vi "set Swept SA - Marker.vi"(6 "On?":bool, 8 "error in (no error)":errorcluster, 9 "trace":i32, 10 "Index":i32, 11 "Keysight 9020A in":refnum<class "Keysight 9020A.lvclass">) -> (0 "error out":errorcluster, 3 "Keysight 9020A out":refnum<class "Keysight 9020A.lvclass">)   [LabVIEW 2023, in "Spectrum Analyzer.lvlib" / "Keysight 9020A.lvclass"]
uses:
  Keysight 9020A.lvclass
  Keysight 9020A.lvclass/Keysight 9020A.ctl
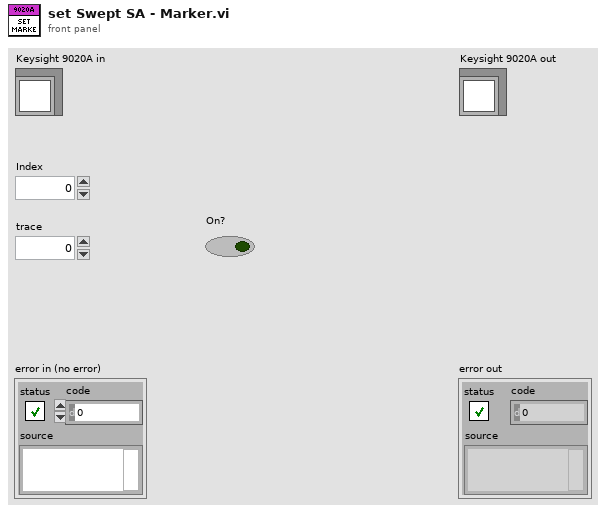
[diagram p1: front panel]
types:
  T1 = typedef "Spectrum Analyzer.lvlib/TYPE Measurement Preset.ctl" = enum16{"Sweep SA Mode", "Channel Power", "Occupied BW", "ACP", "Spurious Emission", "Spurious Emission Mask", "Burst Power (Transmit Power)"}
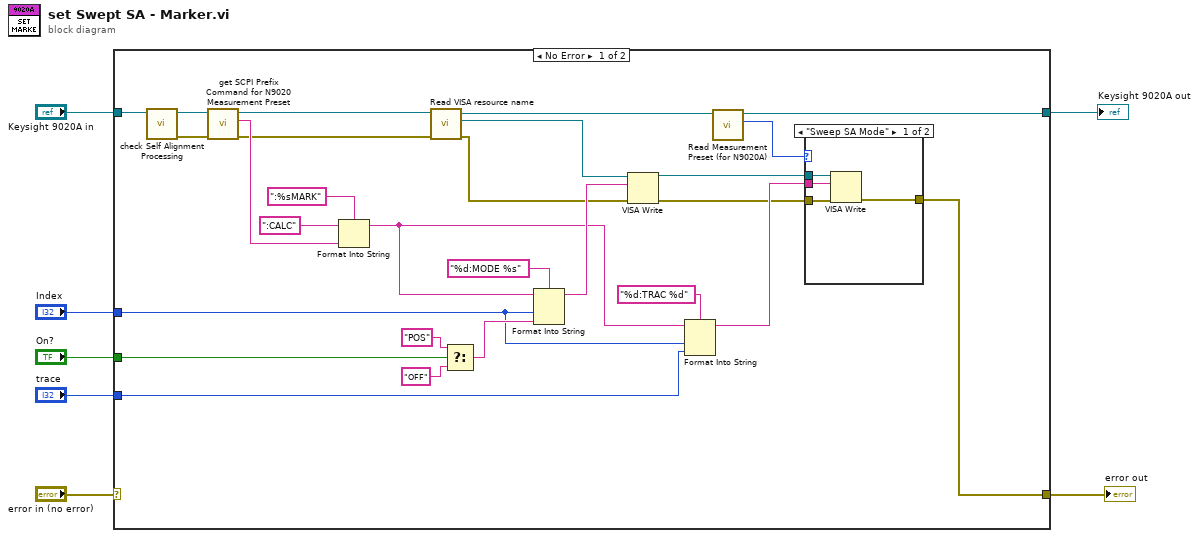
[diagram p0: block diagram]
diagram:
  n1 = case shown="No Error" "error in (no error)" {
    selector: "error in (no error)" -> [_ w40]
    tunnel: "Keysight 9020A in" -> [w12 w41]
    tunnel: [w14 w41] -> w6
    tunnel: [w22 w40] -> w4
    tunnel: "Index" -> [w26 _]
    tunnel: "On?" -> [w32 _]
    tunnel: "trace" -> [w25 _]
    frame No Error {
      n2 = call "check Self Alignment Processing.vi"("Keysight 9020A in"=w12) -> ("error out"=w10:errorcluster, "Keysight 9020A out"=w11:refnum<class "Keysight 9020A.lvclass">)  [unwired: 8 in, 1 out]
      n3 = call "get SCPI Prefix Command for N9020 Measurement Preset.vi"("error in (no error)"=w10, "Keysight 9020A in"=w11) -> ("error out"=w9:errorcluster, "SCPI Prefix Command"=w18:string, "Keysight 9020A out"=w17:refnum<class "Keysight 9020A.lvclass">)  [unwired: 7 in]
      n4 = Format Into String(format string=":%sMARK", initial string=":CALC", w18) -> (resulting string=w16:string)  [unwired: 1 in, 1 out]
      n5 = call "Read VISA resource name.vi"("error in (no error)"=w9, "Keysight 9020A in"=w17) -> ("error out"=w8:errorcluster, "VISA resource name"=w21:refnum<visa-resource-name>, "Keysight 9020A out"=w15:refnum<class "Keysight 9020A.lvclass">)  [unwired: 7 in]
      n6 = Select(t="POS", s=w32, f="OFF") -> (s? t:f=w29:string)
      n7 = Format Into String(format string="%d:MODE %s", initial string=w16, w26, w29) -> (resulting string=w34:string)  [unwired: 1 in, 1 out]
      n8 = VISA Write(VISA resource name=w21, write buffer=w34, error in (no error)=w8) -> (VISA resource name out=w28:refnum<visa-resource-name>, error out=w23:errorcluster)  [unwired: 1 out]
      n9 = Format Into String(format string="%d:TRAC %d", initial string=w16, w26, w25) -> (resulting string=w24:string)  [unwired: 1 in, 1 out]
      n10 = call "Read Measurement Preset (for N9020A).vi"("Keysight 9020A in"=w15) -> ("Measurement Preset"=w13:T1, "Keysight 9020A out"=w14:refnum<class "Keysight 9020A.lvclass">)  [unwired: 8 in, 1 out]
      n11 = case shown="\"Sweep SA Mode\"" w13 {
        tunnel: w28 -> [w38 _]
        tunnel: w24 -> [w37 _]
        tunnel: w23 -> [w36 w39]
        tunnel: [w35 w39] -> w22
        frame "Sweep SA Mode" {
          n12 = VISA Write(VISA resource name=w38, write buffer=w37, error in (no error)=w36) -> (error out=w35:errorcluster)  [unwired: 2 out]
        }
        frame Default {
        }
      }
    }
    frame Error {
    }
  }
  "error out" <- w4
  "Keysight 9020A out" <- w6
